vi "New Time Entry.vi"(7 "Time Entry Store in":refnum<class "Time Entry Store.lvclass">, 8 "error in (no error)":errorcluster, 11 "Time Entry":T1) -> (0 "error out":errorcluster, 3 "New Time Entry":T1, 5 "Time Entry Store out":refnum<class "Time Entry Store.lvclass">)   [LabVIEW 2024, in "Time Entry Store.lvclass"]
doc: "Returns the given time entry with a new GUID in its ID - use it to create an entry before Save Entry. All other fields are passed through unchanged.\n\nGenerated by: Claude"
uses:
  Time Entry Store.lvclass
  Rows/Time Entry.ctl
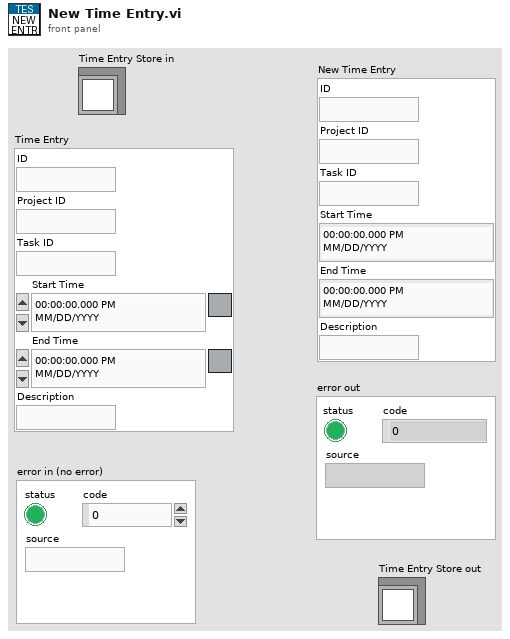
[diagram p1: front panel]
types:
  T1 = typedef "Time Entry.ctl" = cluster{"ID":string, "Project ID":string, "Task ID":string, "Start Time":timestamp, "End Time":timestamp, "Description":string}
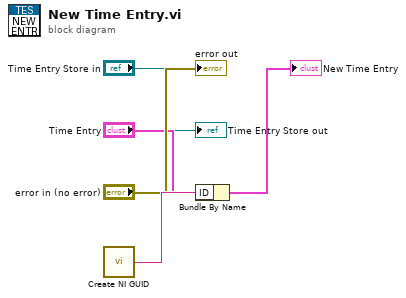
[diagram p0: block diagram]
diagram:
  n1 = call <vilib>:"Create NI GUID.vi"() -> ("NI GUID"=w4:string)
  n2 = Bundle By Name(cluster="Time Entry", "ID"=w4) -> (→"New Time Entry":T1)
  "error out" <- "error in (no error)"
  "Time Entry Store out" <- "Time Entry Store in"
